vi "analiza_vibracija.vi"() -> ()   [LabVIEW 2014]
uses:
  <vilib>/express/express analysis/Spectral/Block/exnSpectralBlock spectral measurements peak poly.vi
  <vilib>/express/express analysis/Spectral/Block/exnSpectralBlock spectral measurements peak DDT.vi
  <vilib>/express/express analysis/Spectral/XNode/ExpressSpectralMeasurementsBlockNode.xnode
panel:
  out "System satus":string
  in  "RMS Threshold [g]":dbl
  out "Peak_to_Peak [g]":dbl
  in  "Sample rate [Hz]":dbl
  in  "Samples to read":dbl
  out "Dominantna frekvencija [Hz]":i32
  out "RMS Vibracije [g]":dbl
  out "Vibracije frekvencijski domen":dynamicdata(graph)
  out "Vibracije vremenski domen":dynamicdata(graph)
  in  "stop (F)":bool
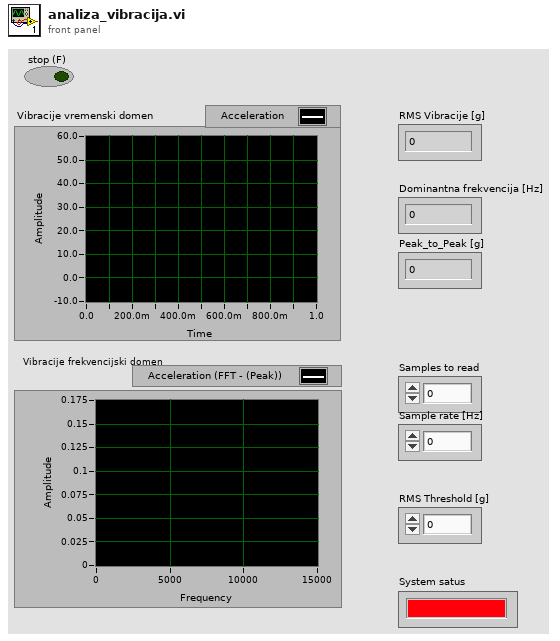
[diagram p1: front panel]
types:
  T1 = cluster{"averaging mode":u16, "weighting mode":u16, "number of averages":u32}
  T2 = cluster{"dB On (F)":bool, "unwrap phase (F)":bool, "convert to degree (F)":bool}
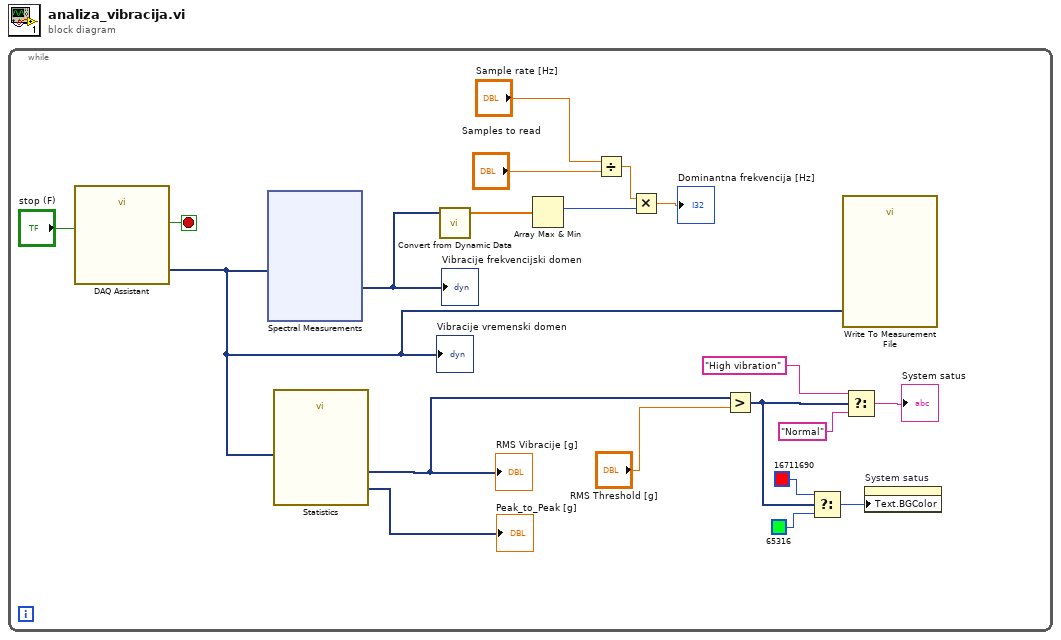
[diagram p0: block diagram]
diagram:
  n1 = while {
    stop <- w19 stop-if-true
    n2 = call "DAQ Assistant"("stop (F)"="stop (F)") -> ("data"=w5:dynamicdata, "stopped"=w19:bool)  [unwired: 15 in, 2 out]
    "Vibracije vremenski domen" <- w5
    n3 = xnode "Spectral Measurements"("Signals"=w5) -> ("FFT - (Peak)"=w18:dynamicdata)  [unwired: 1 in, 2 out]
    "Vibracije frekvencijski domen" <- w18
    n4 = call "Statistics"("Signals"=w5) -> ("RMS"=w4:dynamicdata, "Range"=→"Peak_to_Peak [g]":dynamicdata)  [unwired: 24 in, 1 out]
    "RMS Vibracije [g]" <- w4
    n5 = call "Convert from Dynamic Data"("Dynamic Data Type"=w18) -> ("Array"=w17:dbl[])  [unwired: 3 in]
    n6 = Array Max & Min(array=w17) -> (max index (indices)=w16:i32)  [unwired: 3 out]
    n7 = Divide(x="Sample rate [Hz]", y="Samples to read") -> (x/y=w15:dbl)
    n8 = Multiply(x=w15, y=w16) -> (x*y=→"Dominantna frekvencija [Hz]":dbl)
    n9 = Greater?(x=w4, y="RMS Threshold [g]") -> (0:w9:dynamicdata)
    n10 = Select(t=u32 16711690, s=w9, f=u32 65316) -> (s? t:f=w6:u32)
    n11 = call "Write To Measurement File"("Signals"=w5) -> ()  [unwired: 16 in, 3 out]
    n12 = Select(t="High vibration", s=w9, f="Normal") -> (s? t:f=→"System satus":string)
    n13 = property on="System satus" class="Str"("Text.BGColor"=w6) -> ()  [unwired: 2 in, 2 out]
  }
